vi "TblWrtGlobal (SubVI).vi"(8 "error in":errorcluster, 10 "TblParam0":sgl[][](array[numeric]), 11 "TblParam1":sgl[][](array[numeric])) -> (0 "error out":errorcluster)   [LabVIEW 2017]
uses:
  Global_SNK3_HF.vi
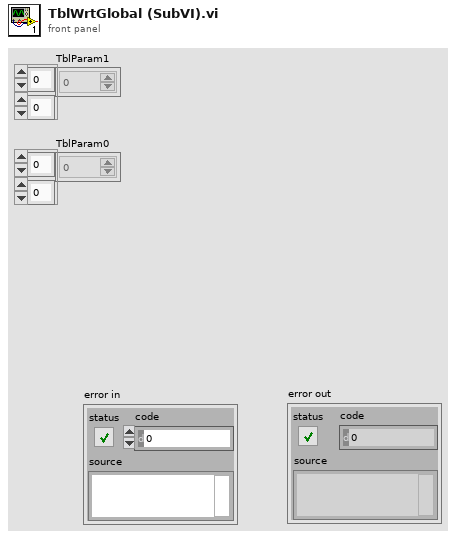
[diagram p1: front panel]
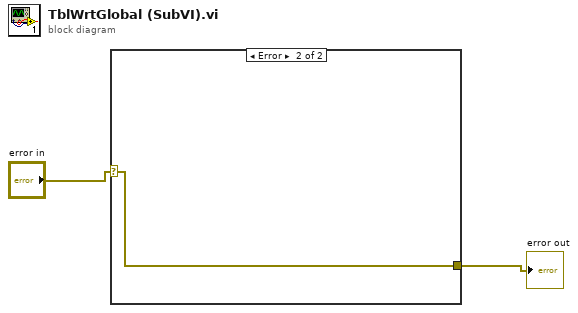
[diagram p0: block diagram]
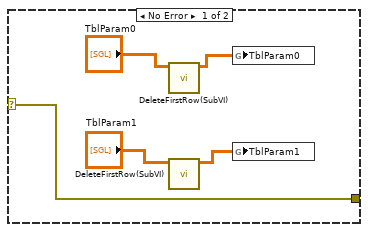
[diagram p2: hidden frame]
diagram:
  n1 = case shown="Error" "error in" {
    selector: "error in" -> [w3 w8]
    tunnel: [w3 w8] -> w1
    frame No Error {
      n2 = call "DeleteFirstRow(SubVI).vi"("TblParam in"="TblParam0") -> ("TblParam out"=w6:sgl[][])  [unwired: 10 in]
      n3 = call "DeleteFirstRow(SubVI).vi"("TblParam in"="TblParam1") -> ("TblParam out"=w7:sgl[][])  [unwired: 10 in]
      n4 = global write "Global_SNK3_HF.vi" "TblParam0"(w6) -> ()
      n5 = global write "Global_SNK3_HF.vi" "TblParam1"(w7) -> ()
    }
    frame Error {
    }
  }
  "error out" <- w1
